vi "Find Wire Segment.vi"(8 "Error":errorcluster, 9 "Co-ordinates":cluster{"x":i16, "y":i16}, 11 "Wire Refnum":refnum<vi>) -> (0 "Error Out":errorcluster, 1 "Downstream Sinks Out":refnum<vi>[](array[refnum]), 2 "Source Node Out":refnum<vi>, 3 "Wire Refnum Out":refnum<vi>)   [LabVIEW 2012, in "Scripting Tools.lvlib"]
doc: "Given a wire refnum and the co-ordinates of a point, finds the terminals that are downstream of the point. Useful for inserting things in a multi-branch wire."
uses:
  Scripting Tools.lvlib
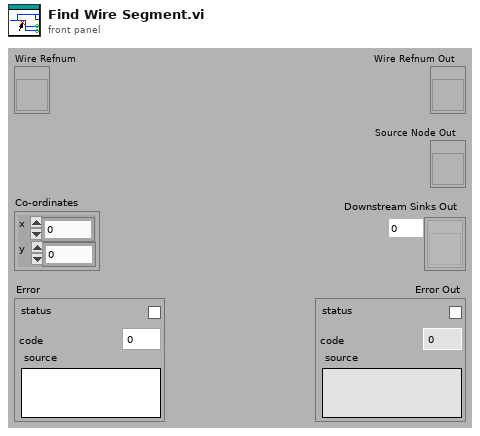
[diagram p1: front panel]
types:
  T1 = cluster{"Position":cluster{"h":i16, "v":i16}, "Flags":i32, "Type":enum32{"LooseEnd", "Endpoint", "Bend", "Junction"}, "Up Joint Index":i16, "Down Joint Index":i16, "Left Joint Index":i16, "Right Joint Index":i16}[]
  T2 = typedef "Scripting Tools.lvlib/Wire Segment Descriptor Type.ctl" = cluster{"Start Position":cluster{"h":i16, "v":i16}, "Finish Position":cluster{"h":i16, "v":i16}, "Start Index":i32, "Finish Index Index":i32, "Start":bool, "Finish":bool, "Direction":u16, "Terminal":refnum<vi>}
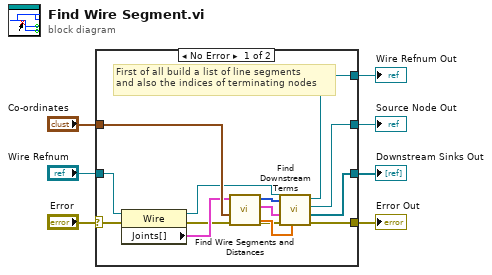
[diagram p0: block diagram]
diagram:
  n1 = case shown="No Error" "Error" {
    selector: "Error" -> [w8 w23]
    tunnel: "Wire Refnum" -> [w21 w22]
    tunnel: "Co-ordinates" -> [w20 _]
    tunnel: [w16 _] -> w5
    tunnel: [w14 w23] -> w3
    tunnel: [w13 _] -> w2
    tunnel: [w11 w22] -> w1
    frame No Error {
      # "First of all build a list of line segments\nand also the indices of terminating nodes"
      n2 = property class="Wire"(reference=w21, error in=w8) -> (reference out=w12:refnum<vi>, error out=w10:errorcluster, "Joints[]"=w15:T1)
      n3 = call "Find Wire Segments and Distances.vi"("Error"=w10, "Co-ordinates"=w20, "Joints[]"=w15) -> ("Error Out"=w9:errorcluster, "Distances"=w19:dbl[], "Segments"=w18:T2[], "Terminating Joints"=w17:i32[])  [unwired: 5 out]
      n4 = call "Find Downstream Terms.vi"("Distances"=w19, "Error"=w9, "Segment Descriptors"=w18, "Terminal Joint Indices"=w17, "Wire Refnum"=w12) -> ("Error Out"=w14:errorcluster, "Array Out"=w16:refnum<vi>[], "Source Node Out"=w13:refnum<vi>, "Wire Refnum Out"=w11:refnum<vi>)  [unwired: 1 in, 2 out]
    }
    frame Error {
    }
  }
  "Error Out" <- w3
  "Downstream Sinks Out" <- w5
  "Wire Refnum Out" <- w1
  "Source Node Out" <- w2
